vi "KeyboardSerializer.vi"(11 "Sample Number":u32) -> (2 "Keyboard No Op":bool, 3 "SerializedKeyPress":T1)   [LabVIEW 2026, in "Core.lvlib"]
uses:
  modules/coordinator/src/Libraries/Core/Core.lvlib
  modules/coordinator/src/Libraries/KeyboardLUTSelector.ctl
  <userlib>/_OpenG.lib/boolean/boolean.llb/openg_boolean__ogtk.lvlib
  <userlib>/_OpenG.lib/comparison/comparison.llb/openg_comparison__ogtk.lvlib
  SerializedKeyPress.ctl
  <userlib>/_OpenG.lib/comparison/comparison.llb/I16 Changed__ogtk.vi
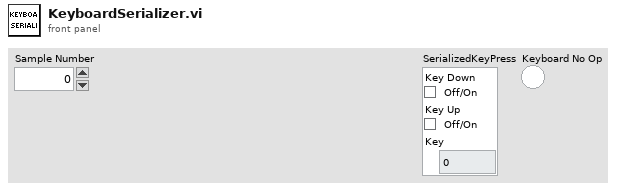
[diagram p1: front panel]
types:
  T1 = typedef "Core.lvlib/SerializedKeyPress.ctl" = cluster{"Key Down":bool, "Key Up":bool, "Key":enum16{"0", "1", "2", "3", "4", "5", "6", "7", "8", "9", "A", "B", "C", "D", "E", "F", "G", "H", "I", "J", "K", "L", "M", "N", "O", "P", "Q", "R", "S", "T", "U", "V", "W", "X", "Y", "Z", "F1", "F2", "F3", "F4", "F5", "F6", "F7", "F8", "F9", "F10", "F11", "F12", "F13", "F14", "F15", "ADD", "BACK", "BACKSLASH", "CAPITAL", "COMMA", "DECIMAL", "DELETE", "DIVIDE", "DOWN", "END", "EQUALS", "ESCAPE", "GRAVE (`)", "HOME", "INSERT", "LBRACKET", "LCONTROL", "LEFT", "L ALT", "LSHIFT", "LWIN", "MINUS", "MULTIPLY", "NEXT", "NUMLOCK", "NUMPAD_0", "NUMPAD_1", "NUMPAD_2", "NUMPAD_3", "NUMPAD_4", "NUMPAD_5", "NUMPAD_6", "NUMPAD_7", "NUMPAD_8", "NUMPAD_9", "PAUSE", "PERIOD", "PRIOR (PG UP)", "RBRACKET", "RCONTROL", "RETURN", "RIGHT", "R ALT", "RSHIFT", "RWIN", "SCROLL", "SEMICOLON", "SLASH", "SPACE", "SUBTRACT", "TAB", "UP", "ENTER (num pad)", "' (quote)"}}
  T2 = typedef "Core.lvlib/KeyboardLUTSelector.ctl" = enum16{"Initialize", "Get Keyboards Keys Pressed at Sample Number", "Assign Keyboard Key Press to Sample Number"}
  T3 = enum16{"0", "1", "2", "3", "4", "5", "6", "7", "8", "9", "A", "B", "C", "D", "E", "F", "G", "H", "I", "J", "K", "L", "M", "N", "O", "P", "Q", "R", "S", "T", "U", "V", "W", "X", "Y", "Z", "F1", "F2", "F3", "F4", "F5", "F6", "F7", "F8", "F9", "F10", "F11", "F12", "F13", "F14", "F15", "ADD", "BACK", "BACKSLASH", "CAPITAL", "COMMA", "DECIMAL", "DELETE", "DIVIDE", "DOWN", "END", "EQUALS", "ESCAPE", "GRAVE (`)", "HOME", "INSERT", "LBRACKET", "LCONTROL", "LEFT", "L ALT", "LSHIFT", "LWIN", "MINUS", "MULTIPLY", "NEXT", "NUMLOCK", "NUMPAD_0", "NUMPAD_1", "NUMPAD_2", "NUMPAD_3", "NUMPAD_4", "NUMPAD_5", "NUMPAD_6", "NUMPAD_7", "NUMPAD_8", "NUMPAD_9", "PAUSE", "PERIOD", "PRIOR (PG UP)", "RBRACKET", "RCONTROL", "RETURN", "RIGHT", "R ALT", "RSHIFT", "RWIN", "SCROLL", "SEMICOLON", "SLASH", "SPACE", "SUBTRACT", "TAB", "UP", "ENTER (num pad)", "' (quote)"}[]
  T4 = enum16{"0", "1", "2", "3", "4", "5", "6", "7", "8", "9", "A", "B", "C", "D", "E", "F", "G", "H", "I", "J", "K", "L", "M", "N", "O", "P", "Q", "R", "S", "T", "U", "V", "W", "X", "Y", "Z", "F1", "F2", "F3", "F4", "F5", "F6", "F7", "F8", "F9", "F10", "F11", "F12", "F13", "F14", "F15", "ADD", "BACK", "BACKSLASH", "CAPITAL", "COMMA", "DECIMAL", "DELETE", "DIVIDE", "DOWN", "END", "EQUALS", "ESCAPE", "GRAVE (`)", "HOME", "INSERT", "LBRACKET", "LCONTROL", "LEFT", "L ALT", "LSHIFT", "LWIN", "MINUS", "MULTIPLY", "NEXT", "NUMLOCK", "NUMPAD_0", "NUMPAD_1", "NUMPAD_2", "NUMPAD_3", "NUMPAD_4", "NUMPAD_5", "NUMPAD_6", "NUMPAD_7", "NUMPAD_8", "NUMPAD_9", "PAUSE", "PERIOD", "PRIOR (PG UP)", "RBRACKET", "RCONTROL", "RETURN", "RIGHT", "R ALT", "RSHIFT", "RWIN", "SCROLL", "SEMICOLON", "SLASH", "SPACE", "SUBTRACT", "TAB", "UP", "ENTER (num pad)", "' (quote)"}
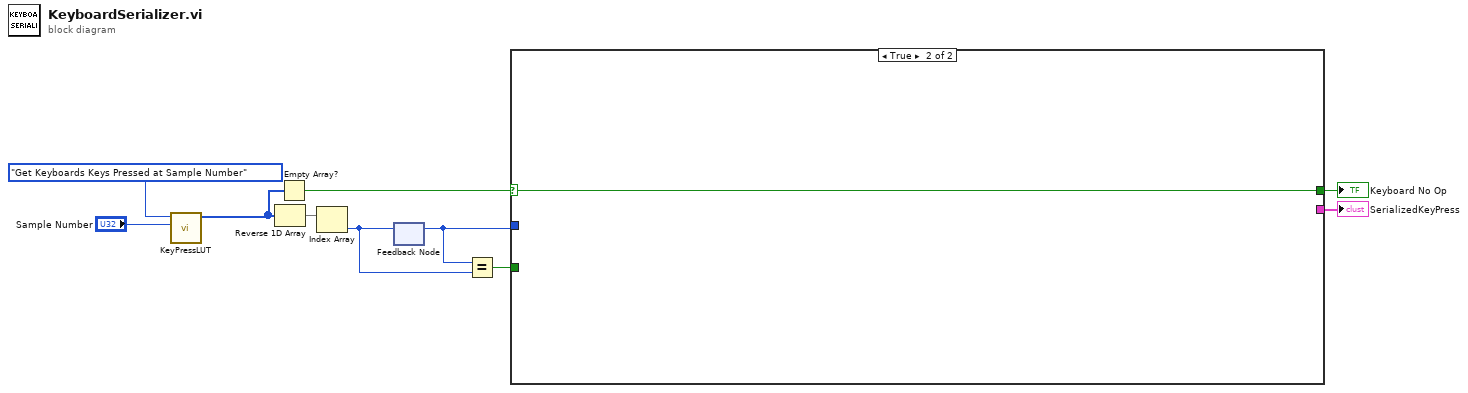
[diagram p0: block diagram]
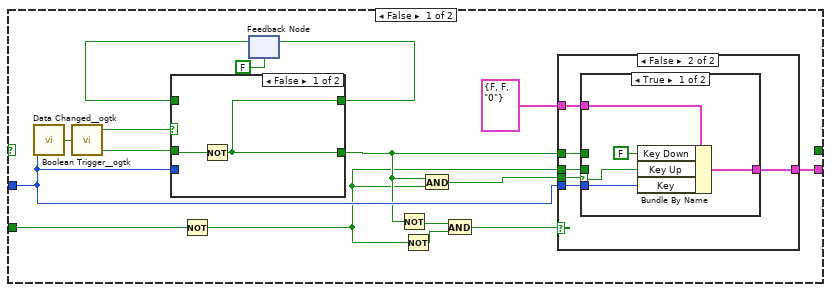
[diagram p2: hidden frame]
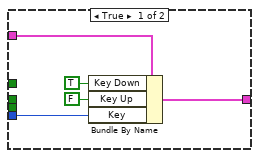
[diagram p3: hidden frame]
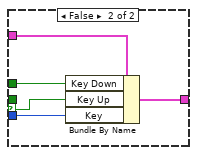
[diagram p4: hidden frame]
diagram:
  n1 = call "KeyPressLUT.vi"("Sample Number"="Sample Number", "LUT Selector"=KeyboardLUTSelector."Get Keyboards Keys Pressed at Sample Number") -> ("KeyboardKeysPressed"=w6:T3)  [unwired: 8 in, 1 out]
  n2 = Reverse 1D Array(array=w6) -> (reversed array=w9:T3)
  n3 = Empty Array?(array=w6) -> (empty?=w7:bool)
  n4 = Index Array(array=w9) -> (element=w3:T4)  [unwired: 1 in]
  n5 = feedback #1() -> (w2:T4)  [unwired: 1 in]
  n6 = feedback-in #1(w3) -> ()
  n7 = Equal?(x=w2, y=w3) -> (x = y?=w8:bool)
  n8 = case shown="True" w7 {
    selector: w7 -> [_ w52]
    tunnel: [w26 _] -> w4
    tunnel: w2 -> [w19 _]
    tunnel: w8 -> [w12 _]
    tunnel: [_ w52] -> w1
    frame False {
      n9 = call-poly <userlib>:"Data Changed__ogtk.vi"("I16"=w19) -> ("Changed"=w25:bool)
      n10 = call <userlib>:"Boolean Trigger__ogtk.vi"("Boolean Input"=w25) -> ("Rising Edge"=w24:bool, "Falling Edge"=w20:bool)  [unwired: 1 in]
      n11 = Not(x=w12) -> (.not. x?=w15:bool)
      n12 = feedback #2(FALSE ("Rising Edge")) -> (w22:bool)
      n13 = case shown="False" w24 {
        selector: w24 -> [_ w51]
        tunnel: w22 -> [_ _]
        tunnel: [w48 w51] -> w21
        tunnel: w19 -> [_ _]
        tunnel: w20 -> [w49 w50]
        tunnel: [w48 w50] -> w17
        frame False {
          n14 = Not(x=w49) -> (.not. x?=w48:bool)
        }
        frame True {
        }
      }
      n15 = feedback-in #2(w21) -> ()
      n16 = Not(x=w17) -> (.not. x?=w16:bool)
      n17 = Not(x=w15) -> (.not. x?=w14:bool)
      n18 = And(x=w17, y=w15) -> (x .and. y?=w18:bool)
      n19 = And(x=w16, y=w14) -> (x .and. y?=w13:bool)
      n20 = case shown="False" w13 {
        tunnel: [w31 w37] -> w26
        tunnel: w19 -> [w30 w36]
        tunnel: w18 -> [_ w35]
        tunnel: w17 -> [_ w34]
        tunnel: w15 -> [_ w33]
        tunnel: T1 {"Key Down"=FALSE, "Key Up"=FALSE, "Key"=enum."0"} -> [w27 w32]
        frame True {
          n21 = Bundle By Name(cluster=w27, "Key Down"=TRUE, "Key Up"=FALSE, "Key"=w30) -> (w31:T1)
        }
        frame False {
          n22 = case shown="True" w35 {
            selector: w35 -> [w39 w45]
            tunnel: [w42 w47] -> w37
            tunnel: w36 -> [w41 w46]
            tunnel: w33 -> [_ _]
            tunnel: w34 -> [_ w44]
            tunnel: w32 -> [w38 w43]
            frame True {
              n23 = Bundle By Name(cluster=w38, "Key Down"=FALSE, "Key Up"=w39, "Key"=w41) -> (w42:T1)
            }
            frame False {
              n24 = Bundle By Name(cluster=w43, "Key Down"=w44, "Key Up"=w45, "Key"=w46) -> (w47:T1)
            }
          }
        }
      }
    }
    frame True {
    }
  }
  "SerializedKeyPress" <- w4
  "Keyboard No Op" <- w1
